vi "FuncVI_Sub - data to spreadsheet string.vi"(4 "delimiter (Tab)":string="\t", 5 "format string":string, 6 "transpose":bool, 7 "data type":T1=enum."DBL Number", 8 "flattened data":string, 9 "dbl":dbl format="%.2f") -> (0 "unflatten error":bool, 3 "spreadsheet string":string)   [LabVIEW 2021]
doc: "::: CalcExpress Toolkit :::\nCopyright (c) 2000-2026 Konstantin Shifershteyn. All rights reserved."
uses:
  cetypes.llb/CalcExpress Data Type.ctl
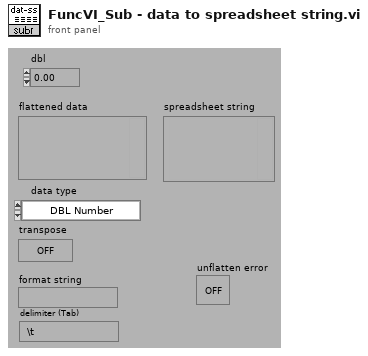
[diagram p1: front panel]
types:
  T1 = typedef "CalcExpress Data Type.ctl" = enum32{"String", "DBL Number", "identifier", "1D Array of DBL", "2D Array of DBL", "CDB Number", "1D Array of CDB", "2D Array of CDB", "1D Array of String", "2D Array of String", "Unknown data type"}
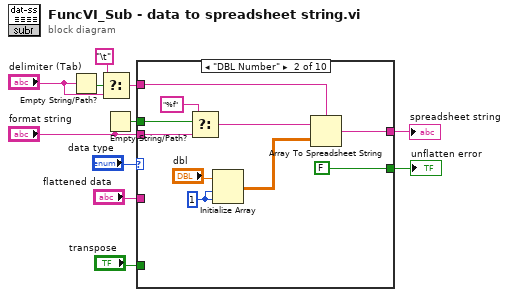
[diagram p0: block diagram]
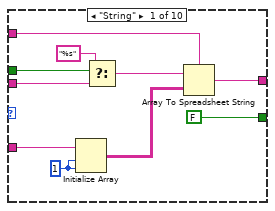
[diagram p2: hidden frame]
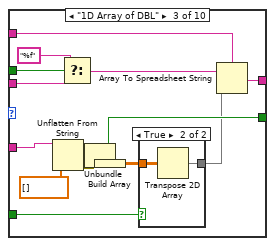
[diagram p3: hidden frame]
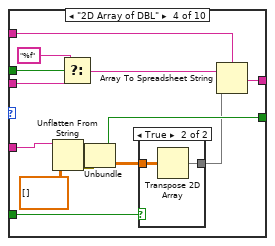
[diagram p5: hidden frame]
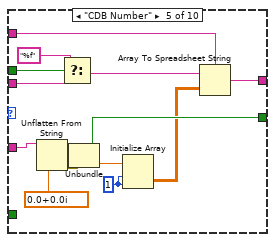
[diagram p7: hidden frame]
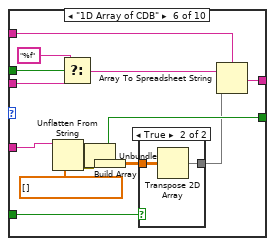
[diagram p8: hidden frame]
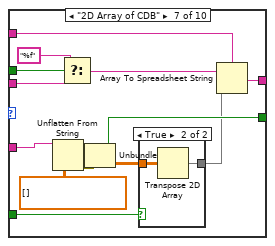
[diagram p10: hidden frame]
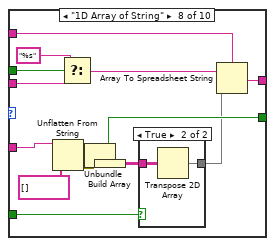
[diagram p12: hidden frame]
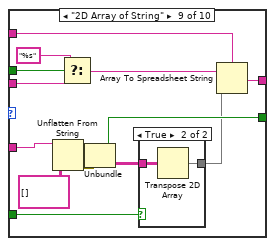
[diagram p14: hidden frame]
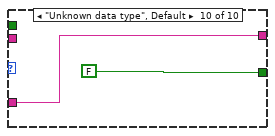
[diagram p16: hidden frame]
diagram:
  n1 = Empty String/Path?(string/path="delimiter (Tab)") -> (empty?=w3:bool)
  n2 = Select(t="\t", s=w3, f="delimiter (Tab)") -> (s? t:f=w4:string)
  n3 = Empty String/Path?(string/path="format string") -> (empty?=w8:bool)
  n4 = case shown="\"DBL Number\"" "data type" {
    tunnel: "flattened data" -> [w14 _ w45 w61 w77 w91 w107 w124 w140 w145]
    tunnel: [w13 w28 w42 w59 w76 w88 w105 w121 w138 w145] -> w7
    tunnel: "format string" -> [w16 w24 w39 w56 w73 w85 w102 w118 w135 _]
    tunnel: [FALSE ("err") FALSE ("err") w41 w58 w75 w87 w104 w120 w137 FALSE ("err")] -> w6
    tunnel: w8 -> [w15 w25 w38 w55 w72 w84 w101 w117 w134 _]
    tunnel: w4 -> [w12 w22 w36 w53 w66 w82 w99 w115 w132 _]
    tunnel: "transpose" -> [_ _ w33 w51 _ w79 w97 w112 w130 _]
    frame "String" {
      w20 = 1
      n5 = Initialize Array(w14, w20, w20) -> (w19:string[][])
      n6 = Select(t="%s" ("format string"), s=w15, f=w16) -> (s? t:f=w17:string)
      n7 = Array To Spreadsheet String(delimiter (Tab)=w12, array=w19, 3:w17) -> (spreadsheet string=w13:string)
    }
    frame "DBL Number" {
      w31 = 1
      n8 = Select(t="%f" ("format string"), s=w25, f=w24) -> (s? t:f=w23:string)
      n9 = Initialize Array("dbl", w31, w31) -> (w29:dbl[][])
      n10 = Array To Spreadsheet String(delimiter (Tab)=w22, array=w29, 3:w23) -> (spreadsheet string=w28:string)
    }
    frame "1D Array of DBL" {
      n11 = Unflatten From String(type=dbl[] [], binary string=w45) -> (value=w43:dbl[], error out=w32:errorcluster)  [unwired: 3 in, 1 out]
      n12 = Select(t="%f" ("format string"), s=w38, f=w39) -> (s? t:f=w40:string)
      n13 = Unbundle(w32) -> ("status"=w41:bool)  [unwired: 2 out]
      n14 = Build Array(w43) -> (w35:dbl[][])
      n15 = case shown="True" w33 {
        tunnel: w35 -> [w46 w48]
        tunnel: [w46 w47] -> w34
        frame False {
        }
        frame True {
          n16 = Transpose 2D Array(2D array=w48) -> (transposed array=w47:dbl[][])
        }
      }
      n17 = Array To Spreadsheet String(delimiter (Tab)=w36, array=w34, 3:w40) -> (spreadsheet string=w42:string)
    }
    frame "2D Array of DBL" {
      n18 = Unflatten From String(type=dbl[][] [], binary string=w61) -> (value=w50:dbl[][], error out=w49:errorcluster)  [unwired: 3 in, 1 out]
      n19 = Select(t="%f" ("format string"), s=w55, f=w56) -> (s? t:f=w57:string)
      n20 = Unbundle(w49) -> ("status"=w58:bool)  [unwired: 2 out]
      n21 = case shown="True" w51 {
        tunnel: w50 -> [w62 w64]
        tunnel: [w62 w63] -> w52
        frame False {
        }
        frame True {
          n22 = Transpose 2D Array(2D array=w64) -> (transposed array=w63:dbl[][])
        }
      }
      n23 = Array To Spreadsheet String(delimiter (Tab)=w53, array=w52, 3:w57) -> (spreadsheet string=w59:string)
    }
    frame "CDB Number" {
      w69 = 1
      n24 = Unflatten From String(type=cdb 0.0+0.0i, binary string=w77) -> (value=w68:cdb, error out=w65:errorcluster)  [unwired: 3 in, 1 out]
      n25 = Select(t="%f" ("format string"), s=w72, f=w73) -> (s? t:f=w74:string)
      n26 = Unbundle(w65) -> ("status"=w75:bool)  [unwired: 2 out]
      n27 = Initialize Array(w68, w69, w69) -> (w67:cdb[][])
      n28 = Array To Spreadsheet String(delimiter (Tab)=w66, array=w67, 3:w74) -> (spreadsheet string=w76:string)
    }
    frame "1D Array of CDB" {
      n29 = Unflatten From String(type=cdb[] [], binary string=w91) -> (value=w89:cdb[], error out=w78:errorcluster)  [unwired: 3 in, 1 out]
      n30 = Select(t="%f" ("format string"), s=w84, f=w85) -> (s? t:f=w86:string)
      n31 = Unbundle(w78) -> ("status"=w87:bool)  [unwired: 2 out]
      n32 = Build Array(w89) -> (w81:cdb[][])
      n33 = case shown="True" w79 {
        tunnel: w81 -> [w92 w94]
        tunnel: [w92 w93] -> w80
        frame False {
        }
        frame True {
          n34 = Transpose 2D Array(2D array=w94) -> (transposed array=w93:cdb[][])
        }
      }
      n35 = Array To Spreadsheet String(delimiter (Tab)=w82, array=w80, 3:w86) -> (spreadsheet string=w88:string)
    }
    frame "2D Array of CDB" {
      n36 = Unflatten From String(type=cdb[][] [], binary string=w107) -> (value=w96:cdb[][], error out=w95:errorcluster)  [unwired: 3 in, 1 out]
      n37 = Select(t="%f" ("format string"), s=w101, f=w102) -> (s? t:f=w103:string)
      n38 = Unbundle(w95) -> ("status"=w104:bool)  [unwired: 2 out]
      n39 = case shown="True" w97 {
        tunnel: w96 -> [w108 w110]
        tunnel: [w108 w109] -> w98
        frame False {
        }
        frame True {
          n40 = Transpose 2D Array(2D array=w110) -> (transposed array=w109:cdb[][])
        }
      }
      n41 = Array To Spreadsheet String(delimiter (Tab)=w99, array=w98, 3:w103) -> (spreadsheet string=w105:string)
    }
    frame "1D Array of String" {
      n42 = Unflatten From String(type=string[] [], binary string=w124) -> (value=w122:string[], error out=w111:errorcluster)  [unwired: 3 in, 1 out]
      n43 = Select(t="%s" ("format string"), s=w117, f=w118) -> (s? t:f=w119:string)
      n44 = Unbundle(w111) -> ("status"=w120:bool)  [unwired: 2 out]
      n45 = Build Array(w122) -> (w114:string[][])
      n46 = case shown="True" w112 {
        tunnel: w114 -> [w125 w127]
        tunnel: [w125 w126] -> w113
        frame False {
        }
        frame True {
          n47 = Transpose 2D Array(2D array=w127) -> (transposed array=w126:string[][])
        }
      }
      n48 = Array To Spreadsheet String(delimiter (Tab)=w115, array=w113, 3:w119) -> (spreadsheet string=w121:string)
    }
    frame "2D Array of String" {
      n49 = Unflatten From String(type=string[][] [], binary string=w140) -> (value=w129:string[][], error out=w128:errorcluster)  [unwired: 3 in, 1 out]
      n50 = Select(t="%s" ("format string"), s=w134, f=w135) -> (s? t:f=w136:string)
      n51 = Unbundle(w128) -> ("status"=w137:bool)  [unwired: 2 out]
      n52 = case shown="True" w130 {
        tunnel: w129 -> [w141 w143]
        tunnel: [w141 w142] -> w131
        frame False {
        }
        frame True {
          n53 = Transpose 2D Array(2D array=w143) -> (transposed array=w142:string[][])
        }
      }
      n54 = Array To Spreadsheet String(delimiter (Tab)=w132, array=w131, 3:w136) -> (spreadsheet string=w138:string)
    }
    frame "Unknown data type", Default {
    }
  }
  "spreadsheet string" <- w7
  "unflatten error" <- w6
